vi "InitFromXML.vi"(8 "error in (no error)":errorcluster, 10 "XML":string, 11 "SystemExec in":refnum<class "SystemExec.lvclass">) -> (0 "error out":errorcluster, 3 "SystemExec out":refnum<class "SystemExec.lvclass">)   [LabVIEW 2023, in "GettingStartedWindow.lvlib" / "SystemExec.lvclass"]
uses:
  <resource>/modes/FRC/Classes/SystemExec/SystemExec.lvclass
  <resource>/modes/FRC/Classes/SystemExec/SystemExec.lvclass/SystemExec.ctl
  <resource>/modes/FRC/Classes/ClickableText/ClickableText.lvclass
  <resource>/modes/FRC/GettingStartedWindow.lvlib
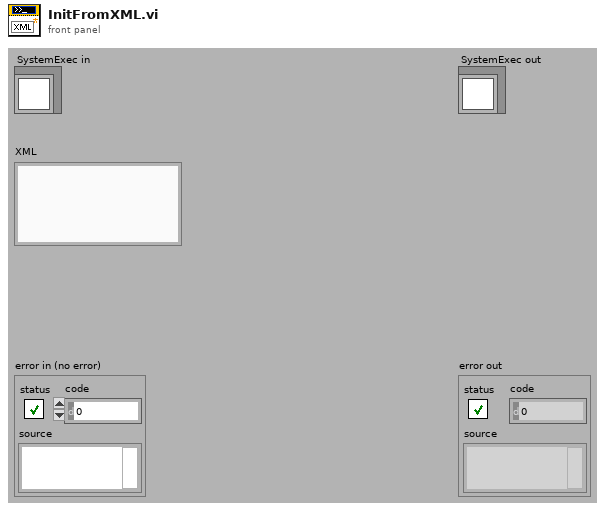
[diagram p1: front panel]
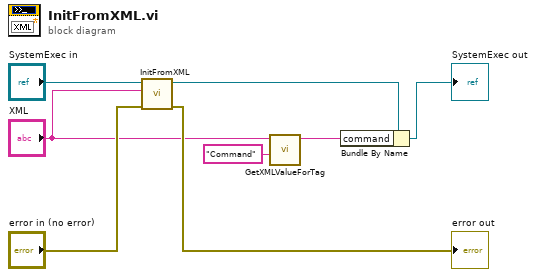
[diagram p0: block diagram]
diagram:
  n1 = call-parent "InitFromXML.vi"("error in (no error)"="error in (no error)", "XML"="XML", "ClickableText in"="SystemExec in") -> ("error out"=→"error out":errorcluster, "ClickableText out"=w3:refnum<class "SystemExec.lvclass">)  [unwired: 7 in]
  n2 = call <resource>:"GetXMLValueForTag.vi"("tag"="Command", "XML"="XML") -> ("value"=w2:string)  [unwired: 8 in, 1 out]
  n3 = Bundle By Name(cluster=w3, "command"=w2) -> (→"SystemExec out":refnum<class "SystemExec.lvclass">)
